vi "XIS Get Frame Number.vi"(8 "error in (no error)":errorcluster) -> (0 "error out":errorcluster, 3 "function return":i32)   [LabVIEW 2025, in "VarexWrapper.lvlib"]
doc: "VAREX_API int XIS_GetFrameNumber();"
uses:
  VarexWrapper.lvlib
  VarexWrapper.dll
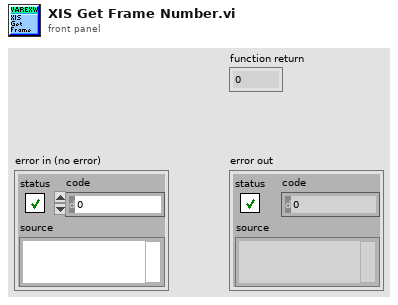
[diagram p1: front panel]
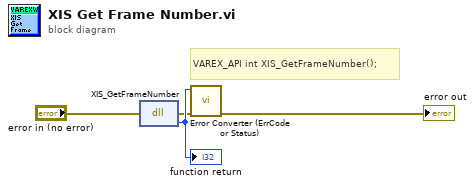
[diagram p0: block diagram]
diagram:
  # "VAREX_API int XIS_GetFrameNumber();"
  n1 = dll-call lib="C:/Users/AriNutpam User/Documents/GitHub/The-Oracle/Image Acquisition/Child Classes/VarexImager/VarexWrapperLvLib/VarexWrapper.*" fn="XIS_GetFrameNumber"(error in="error in (no error)") -> (error out=w2:errorcluster, w4:i32)  [unwired: 2 in, 1 out]
  "function return" <- w4
  n2 = call "Error Converter (ErrCode or Status).vi"("error in (no error)"=w2, "error code"=w4) -> ("error out"=→"error out":errorcluster)  [unwired: 9 in]
